vi "GenerateMenu.vi"(8 "error in":errorcluster, 10 "menu ref in":refnum<k9>, 11 "SystemConfigRepo in":refnum<class "SystemConfigRepo.lvclass">) -> (0 "error out":errorcluster, 2 "menu ref out":refnum<k9>, 3 "SystemConfigRepo out":refnum<class "SystemConfigRepo.lvclass">)   [LabVIEW 2014, in "PL Framework Configuration Tool.lvlib" / "SystemConfigRepo.lvclass"]
uses:
  SystemConfigRepo.lvclass
  <vilib>/Utility/miscctls.llb/LVMenuShortCut.ctl
  <vilib>/NI/Configuration Framework/hierarchy repo/NISE_CEF_HierarchyRepo.lvclass
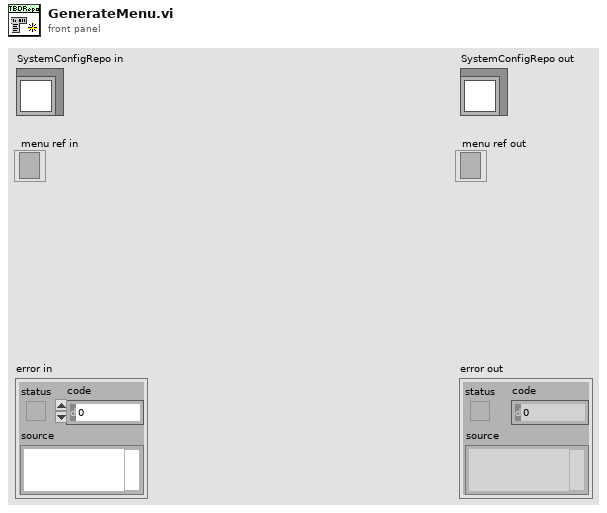
[diagram p1: front panel]
types:
  T1 = typedef "LVMenuShortCut.ctl" = cluster{"Include Shift Key?":bool, "Include Ctrl Key?":bool, "Shortcut Key":string}
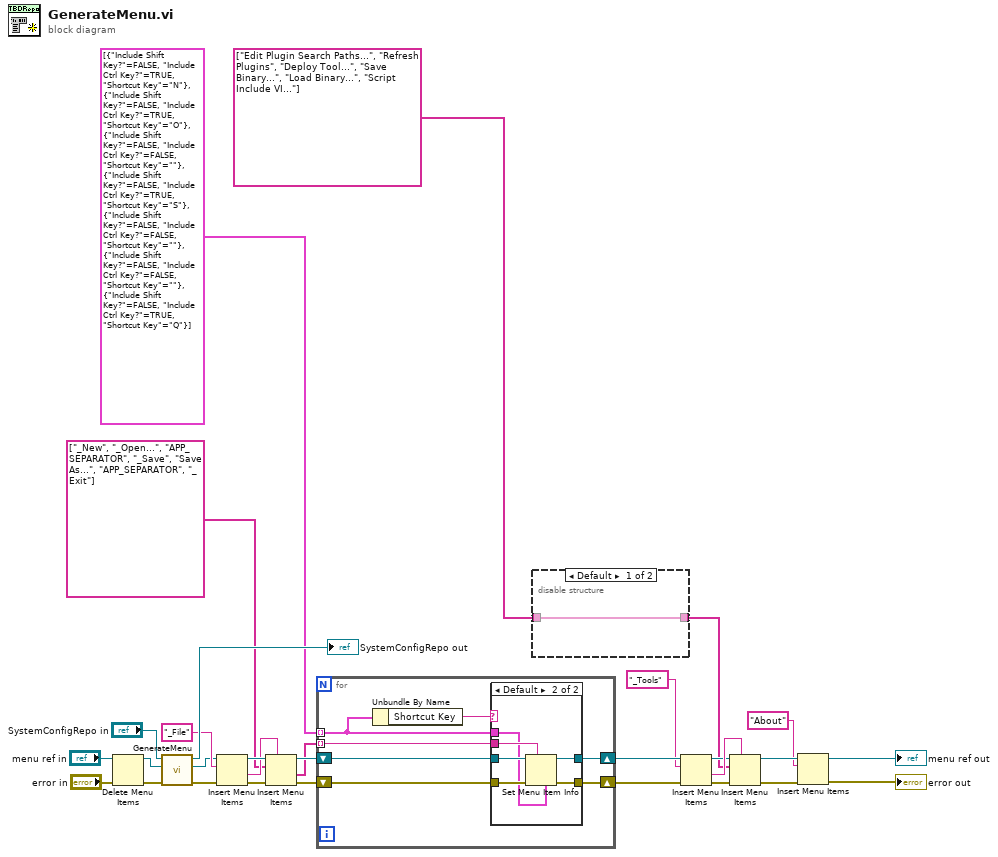
[diagram p0: block diagram]
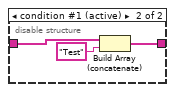
[diagram p2: hidden frame]
diagram:
  n1 = Delete Menu Items(6:"error in", 9:"menu ref in") -> (0:w10:errorcluster, 3:w8:refnum<k9>)  [unwired: 2 in]
  n2 = call-parent "GenerateMenu.vi"("error in"=w10, "menu ref in"=w8, "NISE_CEF_Repository in"="SystemConfigRepo in") -> ("error out"=w7:errorcluster, "menu ref out"=w6:refnum<k9>, "NISE_CEF_Repository out"=→"SystemConfigRepo out":refnum<class "SystemConfigRepo.lvclass">)  [unwired: 6 in]
  n3 = Insert Menu Items(6:w7, 8:"_File", 9:w6) -> (0:w24:errorcluster, 1:w25:string, 3:w26:refnum<k9>)  [unwired: 3 in]
  n4 = Insert Menu Items(5:w25, 6:w24, 8:string[] ["_New", "_Open...", "APP_SEPARATOR", "_Save", "Save As...", "APP_SEPARATOR", "_Exit"] ("item names"), 9:w26) -> (0:w21:errorcluster, 1:w20:string[], 3:w22:refnum<k9>)  [unwired: 2 in]
  n5 = for {
    shift-right: [w35] -> w18
    shift-left: w22 -> [w37]
    tunnel: w20 -> [w34] mode=indexing
    tunnel: T1[] [{"Include Shift Key?"=FALSE, "Include Ctrl Key?"=TRUE, "Shortcut Key"="N"}, {"Include Shift Key?"=FALSE, "Include Ctrl Key?"=TRUE, "Shortcut Key"="O"}, {"Include Shift Key?"=FALSE, "Include Ctrl Key?"=FALSE, "Shortcut Key"=""}, {"Include Shift Key?"=FALSE, "Include Ctrl Key?"=TRUE, "Shortcut Key"="S"}, {"Include Shift Key?"=FALSE, "Include Ctrl Key?"=FALSE, "Shortcut Key"=""}, {"Include Shift Key?"=FALSE, "Include Ctrl Key?"=FALSE, "Shortcut Key"=""}, {"Include Shift Key?"=FALSE, "Include Ctrl Key?"=TRUE, "Shortcut Key"="Q"}] -> [w32] mode=indexing
    shift-right: [w33] -> w17
    shift-left: w21 -> [w36]
    n6 = Unbundle By Name(w32) -> ("Shortcut Key"=w31:string)
    n7 = case shown="Default" w31 {
      tunnel: w37 -> [w39 w45]
      tunnel: w36 -> [w38 w44]
      tunnel: [w39 w43] -> w35
      tunnel: w34 -> [_ w42]
      tunnel: [w38 w41] -> w33
      tunnel: w32 -> [_ w40]
      frame "\u0000" {
      }
      frame Default {
        n8 = Set Menu Item Info(4:w40, 7:w42, 8:w44, 11:w45) -> (0:w41:errorcluster, 3:w43:refnum<k9>)  [unwired: 3 in]
      }
    }
  }
  n9 = disable-structure shown="Default" {
    disable-tunnel: [w46 w48] -> w12
    disable-tunnel: string[] ["Edit Plugin Search Paths...", "Refresh Plugins", "Deploy Tool...", "Save Binary...", "Load Binary...", "Script Include VI..."] ("item names") -> [w46 w49]
    frame condition #0 {
    }
    frame condition #1 (active) {
      n10 = Build Array (concatenate)(w49, "Test") -> (w48:string[])
    }
  }
  n11 = Insert Menu Items(6:w17, 8:"_Tools", 9:w18) -> (0:w15:errorcluster, 1:w16:string, 3:w14:refnum<k9>)  [unwired: 3 in]
  n12 = Insert Menu Items(5:w16, 6:w15, 8:w12, 9:w14) -> (0:w4:errorcluster, 3:w5:refnum<k9>)  [unwired: 2 in, 1 out]
  n13 = Insert Menu Items(6:w4, 8:"About", 9:w5) -> (0:→"error out":errorcluster, 3:→"menu ref out":refnum<k9>)  [unwired: 3 in, 1 out]
